vi "Query IDN.vi"(8 "error in (no error)":errorcluster, 11 "CO3000 in":refnum<class "CO3000.lvclass">) -> (0 "error out":errorcluster, 2 "Connected?":bool, 3 "CO3000 out":refnum<class "CO3000.lvclass">)   [LabVIEW 2023, in "Turn Table and Mast.lvlib" / "CO3000.lvclass"]
uses:
  CO3000.lvclass
  CO3000.lvclass/CO3000.ctl
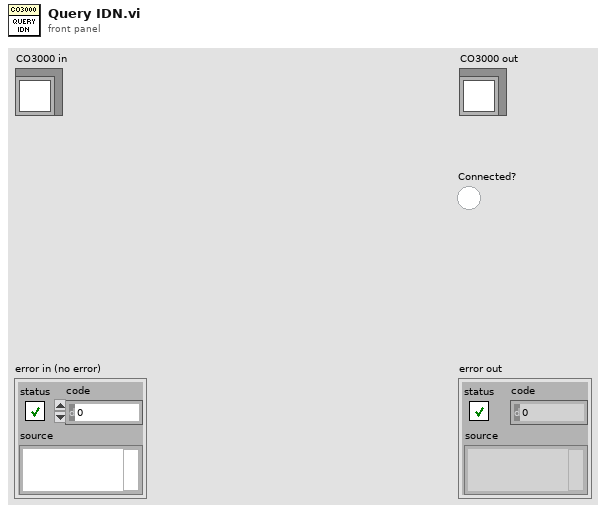
[diagram p1: front panel]
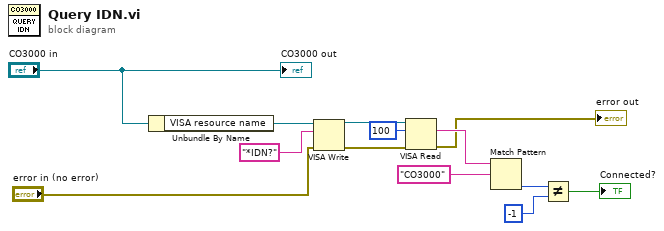
[diagram p0: block diagram]
diagram:
  n1 = Unbundle By Name("CO3000 in") -> ("VISA resource name"=w13:refnum<visa-resource-name>)
  n2 = VISA Write(VISA resource name=w13, write buffer="*IDN?", error in (no error)="error in (no error)") -> (VISA resource name out=w11:refnum<visa-resource-name>, error out=w10:errorcluster)  [unwired: 1 out]
  n3 = VISA Read(VISA resource name=w11, byte count=u32 100, error in (no error)=w10) -> (read buffer=w8:string, error out=→"error out":errorcluster)  [unwired: 2 out]
  n4 = Match Pattern(string=w8, regular expression="CO3000") -> (offset past match=w6:i32)  [unwired: 1 in, 3 out]
  n5 = Not Equal?(x=w6, y=-1) -> (x != y?=→"Connected?":bool)
  "CO3000 out" <- "CO3000 in"
